vi "Enemies_Step.vi"(0 "State":T1={"Tick"=0, "Phase"=0, "PhaseTicks"=0, "Level"=1, "Room"=0, "X10"=0, "Y10"=0, "VY10"=0, "Mode"=0, "Facing"=0, "Run"=0, "Vert"=0, "StandY"=0, "EntryX10"=0, "EntryY10"=0, "EntryMode"=0, "Lives"=4, "Score"=0, "NextLife"=10000, "KeyR"=0, "KeyB"=0, "KeyY"=0, "Torch"=FALSE, "FloorPhase"=0, "Dead"=FALSE, "LevelStart"=FALSE, "Quit"=FALSE, "Sound"=0, "Seed"=12345, "DemoStep"=0, "Tiles"=[], "World"=[], "Enemies"=[], "Highscores"=[], "Name"=[0, 0, 0], "Cursor"=0}, 11 "error in":errorcluster) -> (4 "State out":T1={"Tick"=0, "Phase"=0, "PhaseTicks"=0, "Level"=1, "Room"=0, "X10"=0, "Y10"=0, "VY10"=0, "Mode"=0, "Facing"=0, "Run"=0, "Vert"=0, "StandY"=0, "EntryX10"=0, "EntryY10"=0, "EntryMode"=0, "Lives"=4, "Score"=0, "NextLife"=10000, "KeyR"=0, "KeyB"=0, "KeyY"=0, "Torch"=FALSE, "FloorPhase"=0, "Dead"=FALSE, "LevelStart"=FALSE, "Quit"=FALSE, "Sound"=0, "Seed"=12345, "DemoStep"=0, "Tiles"=[], "World"=[], "Enemies"=[], "Highscores"=[], "Name"=[0, 0, 0], "Cursor"=0}, 15 "error out":errorcluster)   [LabVIEW 2020, in "GH_Engine.lvlib"]
doc: "Moves every enemy by one tick. Snake: stays. Skull: rolls on its floor and turns at walls, doors, edges, ladder holes, vanishing floors and the room edge (Enemy_Walk). Spider: walks like the skull but also over ladder tops; when it passes a ladder or rope it may climb up or down (random), and on reaching a floor it walks on in a random direction (Enemy_Climb). Spiders never leave the room and never jump. Speeds per level (tenths of a pixel per tick). Random numbers from Seed (LCG), one per enemy and tick."
uses:
  GH_Engine.lvlib
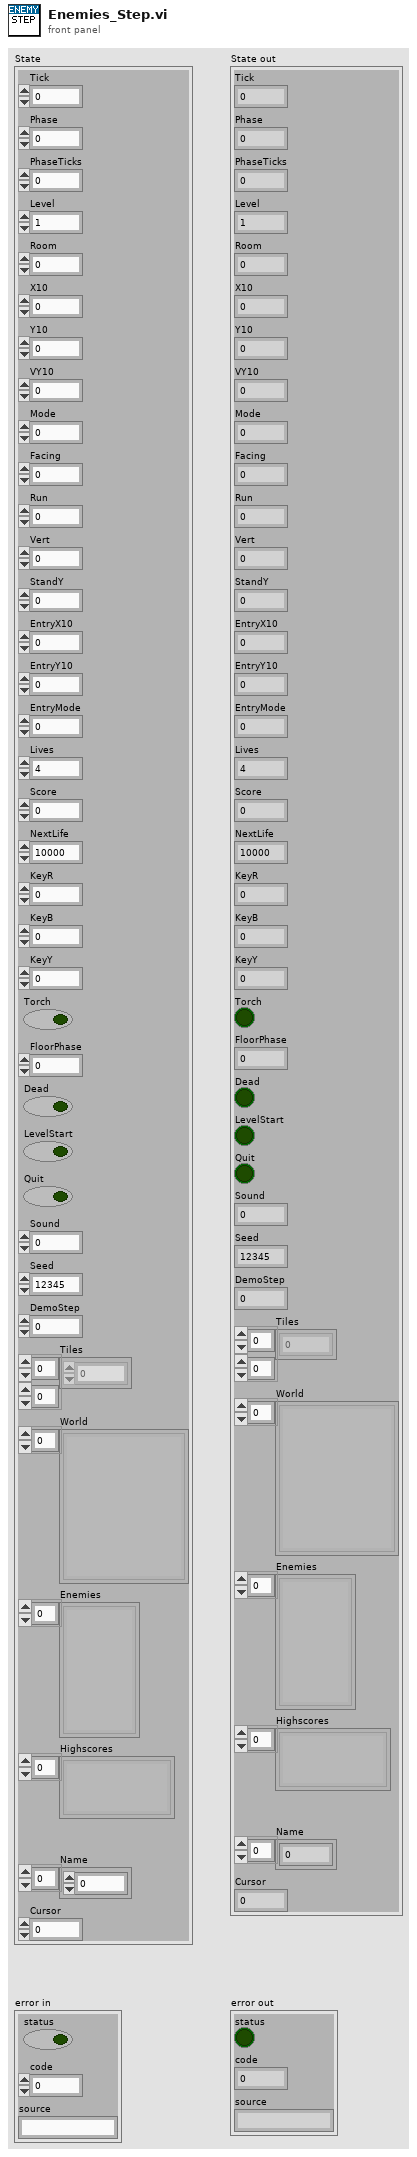
[diagram p1: front panel]
types:
  T1 = cluster{"Tick":u32, "Phase":i32, "PhaseTicks":i32, "Level":i32, "Room":i32, "X10":i32, "Y10":i32, "VY10":i32, "Mode":i32, "Facing":i32, "Run":i32, "Vert":i32, "StandY":i32, "EntryX10":i32, "EntryY10":i32, "EntryMode":i32, "Lives":i32, "Score":i32, "NextLife":i32, "KeyR":i32, "KeyB":i32, "KeyY":i32, "Torch":bool, "FloorPhase":i32, "Dead":bool, "LevelStart":bool, "Quit":bool, "Sound":i32, "Seed":u32, "DemoStep":i32, "Tiles":u8[][], "World":cluster{"ID":string, "Depth":i32, "Column":i32, "Tiles":u8[][]}[], "Enemies":cluster{"Kind":i32, "X10":i32, "Y10":i32, "Dir":i32, "Mode":i32}[], "Highscores":cluster{"Score":i32, "Name":string}[], "Name":i32[], "Cursor":i32}
  T2 = cluster{"Kind":i32, "X10":i32, "Y10":i32, "Dir":i32, "Mode":i32}[]
  T3 = cluster{"Kind":i32, "X10":i32, "Y10":i32, "Dir":i32, "Mode":i32}
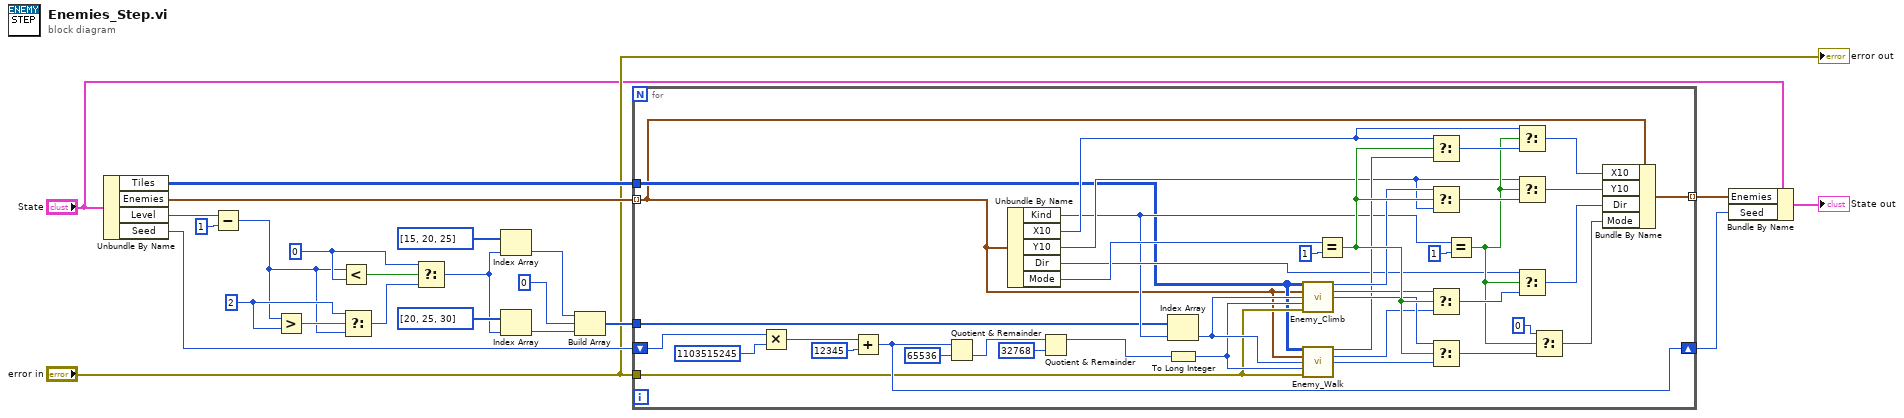
[diagram p0: block diagram]
diagram:
  w10 = 2
  w9 = 0
  n1 = Unbundle By Name("State") -> ("Tiles"=w3:u8[][], "Enemies"=w4:T2, "Level"=w5:i32, "Seed"=w6:u32)
  n2 = Subtract(x=w5, y=1) -> (x-y=w8:i32)
  n3 = Greater?(x=w8, y=w10) -> (0:w12:bool)
  n4 = Less?(x=w8, y=w9) -> (x < y?=w11:bool)
  n5 = Select(t=w10, s=w12, f=w8) -> (s? t:f=w13:i32)
  n6 = Select(t=w9, s=w11, f=w13) -> (s? t:f=w14:i32)
  n7 = Index Array(array=i32[] [15, 20, 25] ("Spider speed"), index=w14) -> (element=w16:i32)
  n8 = Index Array(array=i32[] [20, 25, 30] ("Skull speed"), index=w14) -> (element=w18:i32)
  n9 = Build Array(w16, 0, w18) -> (w20:i32[])
  n10 = for {
    tunnel: "error in" -> [w27]
    tunnel: w4 -> [w24] mode=indexing
    tunnel: w3 -> [w25]
    shift-right: [w29] -> w21
    shift-left: w6 -> [w28]
    tunnel: w20 -> [w26]
    tunnel: [w63] -> w22 mode=indexing
    n11 = Multiply(x=w28, y=u32 1103515245) -> (x*y=w36:u32)
    n12 = Add(x=w36, y=u32 12345) -> (x+y=w29:u32)
    n13 = Quotient & Remainder(x=w29, y=u32 65536) -> (floor(x/y)=w39:u32)  [unwired: 1 out]
    n14 = Unbundle By Name(w24) -> ("Kind"=w30:i32, "X10"=w31:i32, "Y10"=w32:i32, "Dir"=w33:i32, "Mode"=w34:i32)
    n15 = Quotient & Remainder(x=w39, y=u32 32768) -> (x-y*floor(x/y)=w41:u32)  [unwired: 1 out]
    n16 = Index Array(array=w26, index=w30) -> (element=w43:i32)
    n17 = To Long Integer(number=w41) -> (32bit integer=w42:i32)
    n18 = call "Enemy_Climb.vi"("Tiles"=w25, "Enemy"=w24, "Speed"=w43, "Random"=w42, "error in"=w27) -> ("Y10"=w47:i32, "Dir"=w48:i32, "Mode"=w49:i32)  [unwired: 7 in, 1 out]
    n19 = call "Enemy_Walk.vi"("Tiles"=w25, "Enemy"=w24, "Speed"=w43, "Random"=w42, "error in"=w27) -> ("X10"=w44:i32, "Dir"=w45:i32, "Mode"=w46:i32)  [unwired: 7 in, 1 out]
    n20 = Equal?(x=w34, y=1) -> (x = y?=w53:bool)
    n21 = Select(t=w31, s=w53, f=w44) -> (s? t:f=w54:i32)
    n22 = Select(t=w47, s=w53, f=w32) -> (s? t:f=w56:i32)
    n23 = Select(t=w48, s=w53, f=w45) -> (s? t:f=w58:i32)
    n24 = Select(t=w49, s=w53, f=w46) -> (s? t:f=w61:i32)
    n25 = Equal?(x=w30, y=1) -> (x = y?=w51:bool)
    n26 = Select(t=w31, s=w51, f=w54) -> (s? t:f=w55:i32)
    n27 = Select(t=w32, s=w51, f=w56) -> (s? t:f=w57:i32)
    n28 = Select(t=w33, s=w51, f=w58) -> (s? t:f=w59:i32)
    n29 = Select(t=0, s=w51, f=w61) -> (s? t:f=w62:i32)
    n30 = Bundle By Name(cluster=w24, "X10"=w55, "Y10"=w57, "Dir"=w59, "Mode"=w62) -> (w63:T3)
  }
  n31 = Bundle By Name(cluster="State", "Enemies"=w22, "Seed"=w21) -> (→"State out":T1)
  "error out" <- "error in"
